vi "Configuration.vi"() -> ()   [LabVIEW 2023]
panel:
  in  "Max Drive Speed":dbl=17.49
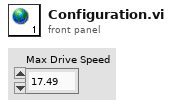
[diagram p1: front panel]
diagram:
